vi "Preprocess_and_Convert_IMAQ_Image_to_Array.vi"(7 "PreProcessing_Options":T2={"DS_Name"="delete", "Input_Dims"={"C"=3, "H"=224, "W"=224}, "Cropping"={"Left"=0.0, "Top"=0.0, "Right"=0.0, "Bottom"=0.0}, "Interpolation Type"=1, "MultiStage_ReSample?"=FALSE, "Dataset_Stats"={"means"={"R"=0.5385, "G"=0.5348, "B"=0.551}, "stds"={"R"=0.3673, "G"=0.3673, "B"=0.3505}}} {"Dataset_Stats"."stds"."R" format="%#_3g"; "Dataset_Stats"."stds"."G" format="%#_3g"; "Dataset_Stats"."stds"."B" format="%#_3g"; "Dataset_Stats"."means"."R" format="%#_3g"; "Dataset_Stats"."means"."G" format="%#_3g"; "Dataset_Stats"."means"."B" format="%#_3g"; "Interpolation Type" items=["Zero Order", "Bi-Linear", "Quadratic", "Cubic Spline"]}, 8 "error in (no error)":errorcluster, 11 "Image In":T1=refnum) -> (0 "error out":errorcluster, 1 "Image_Out(Cropped)":T1, 2 "Norm_Img_Out":sgl[][][](array[numeric]), 3 "Image_Out(PreProcessed)":T1, 5 "dT_Preprocessing":dbl)   [LabVIEW 2020]
uses:
  <vilib>/Ngene/DeepLTK Anomaly Detection Addon/Toolkit/API/Controls/NNPC_PreProcessing_Options.ctl
  <vilib>/Ngene/Deep Learning Toolkit/Toolkit/NN_Data/API/NN_Dims(C,H,W).ctl
  <vilib>/Ngene/DeepLTK Anomaly Detection Addon/Toolkit/API/Controls/Crop_CFG.ctl
  <vilib>/Ngene/DeepLTK Anomaly Detection Addon/Toolkit/API/Controls/NNPC_DS_Stats.ctl
  <vilib>/Ngene/DeepLTK Anomaly Detection Addon/Toolkit/API/Controls/Image_Stats_RGB.ctl
  <vilib>/vision/Image Controls.llb/IMAQ Image.ctl
  512652e7-8bb2-4c08-b1e0-f69a9963c1b4.vi
  1e7322f7-afa4-4f32-9821-a837e705fa4e.vi
  <vilib>/Utility/High Resolution Relative Seconds.vi
  <vilib>/vision/NI_Vision_Development_Module.lvlib
  <vilib>/Ngene/Deep Learning Toolkit/Toolkit/Deep_Learning_Toolkit_by_Ngene.lvlib
  <vilib>/Ngene/DeepLTK Anomaly Detection Addon/Toolkit/DeepLTK_Anomaly_Detection_Addon.lvlib
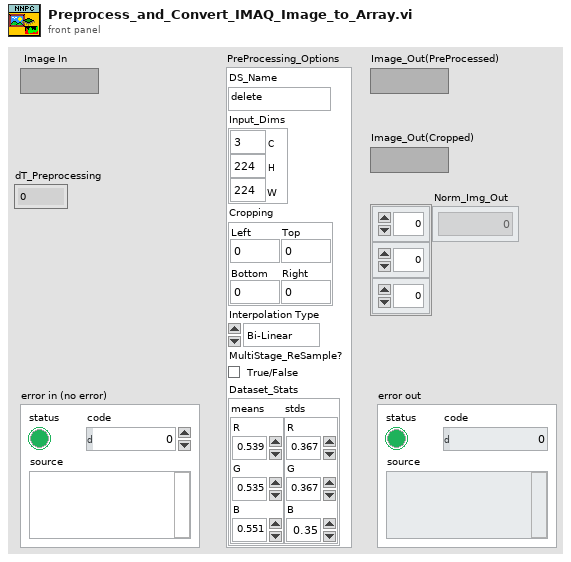
[diagram p1: front panel]
types:
  T1 = typedef "IMAQ Image.ctl" = refnum<image>
  T2 = typedef "DeepLTK_Anomaly_Detection_Addon.lvlib/NNPC_PreProcessing_Options.ctl" = cluster{"DS_Name":string, "Input_Dims":T3, "Cropping":T4, "Interpolation Type":u32, "MultiStage_ReSample?":bool, "Dataset_Stats":T5}
  T3 = typedef "Deep_Learning_Toolkit_by_Ngene.lvlib/NN_Dims(C,H,W).ctl" = cluster{"C":i32, "H":i32, "W":i32}
  T4 = typedef "DeepLTK_Anomaly_Detection_Addon.lvlib/Crop_CFG.ctl" = cluster{"Left":sgl, "Top":sgl, "Right":sgl, "Bottom":sgl}
  T5 = typedef "DeepLTK_Anomaly_Detection_Addon.lvlib/NNPC_DS_Stats.ctl" = cluster{"means":T6, "stds":T6}
  T6 = typedef "DeepLTK_Anomaly_Detection_Addon.lvlib/Image_Stats_RGB.ctl" = cluster{"R":sgl, "G":sgl, "B":sgl}
  T7 = typedef "Image Type" = u32
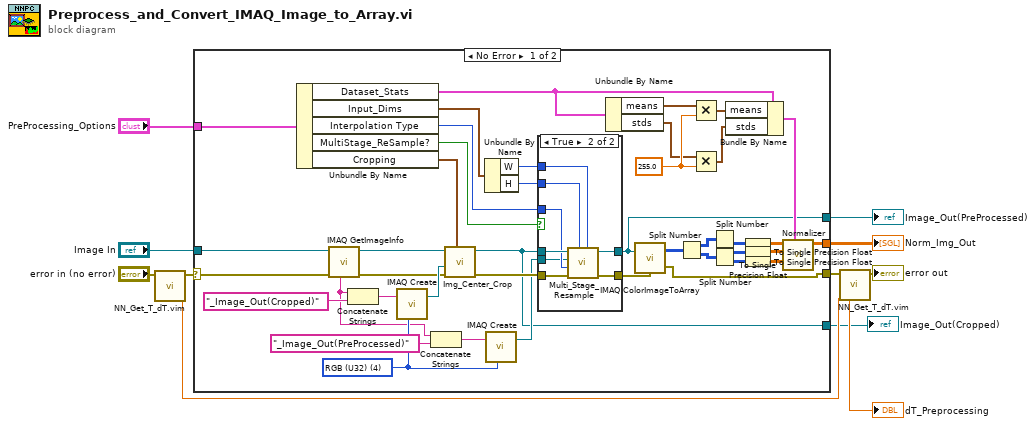
[diagram p0: block diagram]
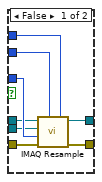
[diagram p2: hidden frame]
diagram:
  n1 = call "NN_Get_T_dT.vim"("error in"="error in (no error)") -> ("T_out"=w4:dbl, "error out"=w5:errorcluster)  [unwired: 6 in, 1 out]
  n2 = case shown="No Error" w5 {
    selector: w5 -> [w13 w68]
    tunnel: "PreProcessing_Options" -> [w51 _]
    tunnel: "Image In" -> [w17 _]
    tunnel: [w30 w68] -> w10
    tunnel: [w29 _] -> w9
    tunnel: [w25 _] -> w2
    tunnel: [w19 _] -> w1
    frame No Error {
      w18 = T7 4 items=["Grayscale (U8)", "Grayscale (I16)", "Grayscale (SGL)", "Complex (CSG)", "RGB (U32)", "HSL (U32)", "RGB (U64)", "Grayscale (U16)"] ("Image Type")
      w43 = sgl 255.0 ("R")
      n3 = Unbundle By Name(w51) -> ("Dataset_Stats"=w44:T5, "Input_Dims"=w34:T3, "Interpolation Type"=w28:u32, "MultiStage_ReSample?"=w27:bool, "Cropping"=w24:T4)
      n4 = call "IMAQ GetImageInfo"("error in (no error)"=w13, "Image"=w17) -> ("error out"=w12:errorcluster, "Image Name"=w14:string)  [unwired: 2 in, 6 out]
      n5 = Concatenate Strings(w14, "_Image_Out(Cropped)" ("Image Name")) -> (w16:string)
      n6 = call "IMAQ Create"("Image Name"=w16, "Image Type"=w18) -> ("New Image"=w21:T1)  [unwired: 3 in, 1 out]
      n7 = Concatenate Strings(w14, "_Image_Out(PreProcessed)" ("Image Name")) -> (w15:string)
      n8 = call "Img_Center_Crop.vi"("Crop_CFG"=w24, "error in"=w12, "Image Dest In"=w21, "Image Src In"=w17) -> ("error out"=w23:errorcluster, "Image Dest Out"=w19:T1)  [unwired: 6 in]
      n9 = Unbundle By Name(w34) -> ("W"=w32:i32, "H"=w31:i32)
      n10 = call "IMAQ Create"("Image Name"=w15, "Image Type"=w18) -> ("New Image"=w20:T1)  [unwired: 3 in, 1 out]
      n11 = case shown="True" w27 {
        tunnel: [w59 w64] -> w33
        tunnel: [w58 w65] -> w25
        tunnel: w28 -> [w57 w61]
        tunnel: w19 -> [w53 w62]
        tunnel: w32 -> [w56 w63]
        tunnel: w31 -> [w55 w66]
        tunnel: w23 -> [w54 w67]
        tunnel: w20 -> [w52 w60]
        frame False {
          n12 = call "IMAQ Resample"("X Resolution"=w56, "Y Resolution"=w55, "error in (no error)"=w54, "Interpolation Type"=w57, "Image Dst"=w52, "Image Src"=w53) -> ("error out"=w59:errorcluster, "Image Dst Out"=w58:T1)  [unwired: 4 in]
        }
        frame True {
          n13 = call "Multi_Stage_Resample.vi"("X Resolution"=w63, "Y Resolution"=w66, "error in"=w67, "Interpolation Type"=w61, "Image Dest In"=w60, "Image Src"=w62) -> ("error out"=w64:errorcluster, "Img out"=w65:T1)  [unwired: 4 in]
        }
      }
      n14 = Unbundle By Name(w44) -> ("means"=w41:T6, "stds"=w42:T6)
      n15 = call "IMAQ ColorImageToArray"("Image"=w25, "error in (no error)"=w33) -> ("Image Pixels (U32)"=w40:u32[][], "error out"=w30:errorcluster)  [unwired: 2 in, 1 out]
      n16 = Split Number(x=w40) -> (hi(x)=w36:u16[][], lo(x)=w35:u16[][])
      n17 = Multiply(x=w41, y=w43) -> (x*y=w46:T6)
      n18 = Multiply(x=w42, y=w43) -> (x*y=w47:T6)
      n19 = Split Number(x=w36) -> (lo(x)=w37:u8[][])  [unwired: 1 out]
      n20 = Split Number(x=w35) -> (hi(x)=w38:u8[][], lo(x)=w39:u8[][])
      n21 = Bundle By Name(cluster=w44, "means"=w46, "stds"=w47) -> (w45:T5)
      n22 = To Single Precision Float(number=w37) -> (single precision float=w48:sgl[][])
      n23 = To Single Precision Float(number=w38) -> (single precision float=w49:sgl[][])
      n24 = To Single Precision Float(number=w39) -> (single precision float=w50:sgl[][])
      n25 = call "Normalizer.vi"("Dataset_Stats"=w45, "B"=w50, "G"=w49, "R"=w48) -> ("Norm_Img_Out"=w29:sgl[][][])  [unwired: 7 in]
    }
    frame Error {
    }
  }
  "Norm_Img_Out" <- w9
  "Image_Out(Cropped)" <- w1
  "Image_Out(PreProcessed)" <- w2
  n26 = call "NN_Get_T_dT.vim"("T_in"=w4, "error in"=w10) -> ("error out"=→"error out":errorcluster, "dT"=→"dT_Preprocessing":dbl)  [unwired: 5 in, 1 out]
